vi "enkoder_lfsr.vi"() -> ()   [LabVIEW 2025]
panel:
  in  "Stop":bool
  in  "D":u32 format="%b"
  out "CRC":u32 format="%b"
  out "Message with CRC":u32 format="%b"
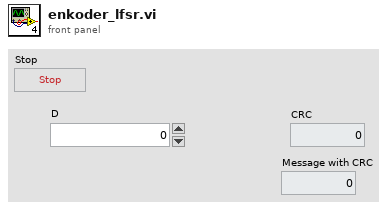
[diagram p1: front panel]
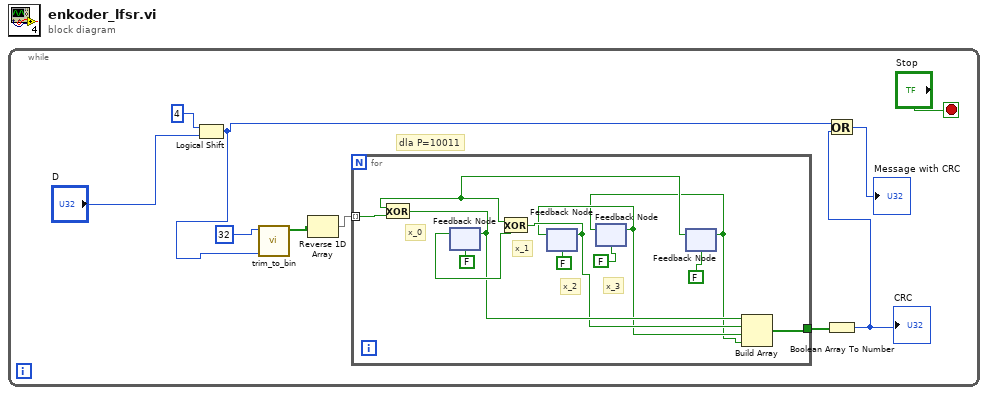
[diagram p0: block diagram]
diagram:
  n1 = while {
    stop <- "Stop" stop-if-true
    # "dla P=10011"
    n2 = Logical Shift(y=i16 4, x="D") -> (x << y=w1:u32)
    n3 = call "trim_to_bin.vi"("number"=w1, "constant"=u32 32) -> ("new array"=w8:bool[])  [unwired: 8 in, 1 out]
    n4 = Reverse 1D Array(array=w8) -> (reversed array=w7:bool[])
    n5 = for {
      tunnel: w7 -> [w22] mode=indexing
      tunnel: [w15] -> w6
      # "x_3"
      # "x_2"
      # "x_1"
      # "x_0"
      n6 = feedback #1(FALSE) -> (w16:bool)
      n7 = feedback #2(FALSE) -> (w12:bool)
      n8 = feedback #3(FALSE) -> (w11:bool)
      n9 = feedback-in #3(w12) -> ()
      n10 = feedback #4(FALSE) -> (w17:bool)
      n11 = Exclusive Or(1:w22, 2:w17) -> (0:w14:bool)
      n12 = feedback-in #1(w14) -> ()
      n13 = Exclusive Or(1:w16, 2:w17) -> (0:w13:bool)
      n14 = feedback-in #2(w13) -> ()
      n15 = feedback-in #4(w11) -> ()
      n16 = Build Array(w14, w13, w12, w11) -> (w15:bool[])
    }
    n17 = Boolean Array To Number(Boolean array=w6) -> (number=w3:u32)
    "CRC" <- w3
    n18 = Or(x=w1, y=w3) -> (x .or. y?=→"Message with CRC":u32)
  }
